vi "Create ToastSource (Poly).vi"   [LabVIEW 2026, in "ToastNotification.lvlib"]
doc: "Select a concrete toast-source creation VI. The current instance, Create ToastBuilder, returns a ToastBuilder for composition and use with ToastService.Show. The caller owns Close. Creation is skipped on incoming error; service initialization and callback registration are separate."
uses:
  ToastNotification.lvlib
  ToastBuilder/ToastBuilder.lvclass
  ToastFromXML/ToastFromXML.lvclass
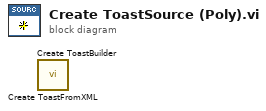
[diagram p0: block diagram]
diagram:
  n1 = call "Create ToastFromXML.vi"() -> ()  [unwired: 10 in, 2 out]
  n2 = call "Create ToastBuilder.vi"() -> ()  [unwired: 10 in, 2 out]
